vi "Translate front panels.vi"(7 "error in (no error)":errorcluster, 9 "Defer Panel Updates? (T)":bool=TRUE, 10 "Language":string) -> (0 "error out":errorcluster)   [LabVIEW 2019, in "Language Selection.lvlib"]
doc: "Translates the controls in the VI according to the translation settings\n- - -\nCopyright (c) 2026, Merecs Engineering GmbH"
uses:
  Language Selection.lvlib
  private/Global Language Selection.vi
panel:
  # "Connector Pane"
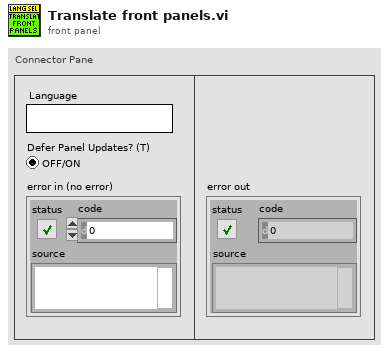
[diagram p1: front panel]
types:
  T1 = typedef "Language Selection.lvlib/Cluster Language Configuration.ctl" = cluster{"Data":T2, "Supported Languages":cluster{"ANSI":string[], "Unicode":string[]}, "VIs":path[], "FP Translations":T3[], "Text Translations":T3[]}
  T2 = typedef "Language Selection.lvlib/Cluster Settings Data.ctl" = cluster{"Startup Language":string, "Default Language":string, "Languages":cluster{"ANSI":string[], "Unicode":string[]}}
  T3 = typedef "Language Selection.lvlib/Cluster Language.ctl" = cluster{"Label":string, "Comment":string, "Property":T4[]}
  T4 = typedef "Language Selection.lvlib/Cluster PropertyTranslation.ctl" = cluster{"Type":T5, "Translation ANSI":string[], "Translation Unicode":string[]}
  T5 = typedef "Language Selection.lvlib/Enum Property Type.ctl" = enum16{"NA", "Caption", "String Value", "Boolean Text", "Ring Strings", "1D Array Elements", "2D Array Elements", "(MC)Listbox Header", "(MC)Listbox Items", "Tab Pages Names", "X & Y GraphChart", "Plot Names", "Table Headers", "Table Items", "TipStrip", "Combobox Strings", "Cursor Name", "Tree Col Headers"}
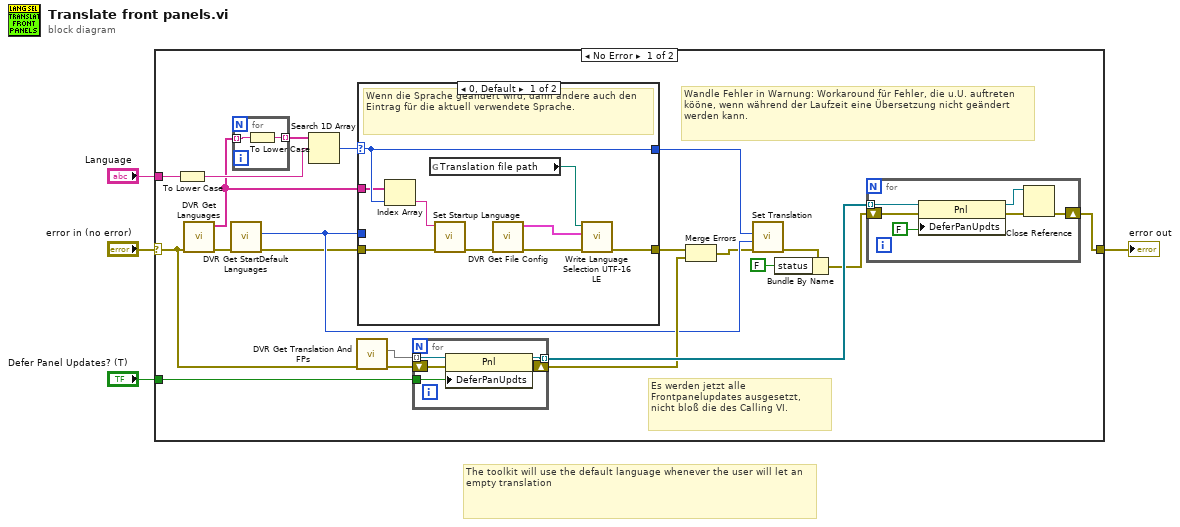
[diagram p0: block diagram]
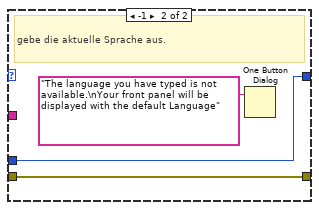
[diagram p2: hidden frame]
diagram:
  # "The toolkit will use the default language whenever the user will let an empty translation"
  n1 = case shown="No Error" "error in (no error)" {
    selector: "error in (no error)" -> [w10 w51]
    tunnel: [w18 w51] -> w3
    tunnel: "Language" -> [w23 _]
    tunnel: "Defer Panel Updates? (T)" -> [w19 _]
    frame No Error {
      # "Es werden jetzt alle Frontpanelupdates ausgesetzt, \nnicht bloß die des Calling VI."
      # "Wandle Fehler in Warnung: Workaround für Fehler, die u.U. auftreten kööne, wenn während der Laufzeit eine Übersetzung nicht geändert werden kann."
      n2 = To Lower Case(string=w23) -> (all lower case string=w22:string)
      n3 = call "DVR Get Languages.vi"("error in (no error)"=w10) -> ("error out"=w12:errorcluster, "Languages"=w14:string[])  [unwired: 7 in, 2 out]
      n4 = call "DVR Get StartDefault Languages.vi"("error in (no error)"=w12) -> ("error out"=w11:errorcluster, "Default"=w13:i32)  [unwired: 8 in, 1 out]
      n5 = for {
        tunnel: w14 -> [w38] mode=indexing
        tunnel: [w37] -> w21 mode=indexing
        n6 = To Lower Case(string=w38) -> (all lower case string=w37:string)
      }
      n7 = Search 1D Array(1D array=w21, element=w22) -> (index of element=w24:i32)  [unwired: 1 in]
      n8 = call "DVR Get Translation And FPs.vi"("error in (no error)"=w10) -> ("error out"=w15:errorcluster, "Front panels"=w16:set{refnum<vi>})  [unwired: 8 in, 1 out]
      n9 = case shown="0, Default" w24 {
        selector: w24 -> [w47 _]
        tunnel: [w47 w48] -> w20
        tunnel: w11 -> [w45 w50]
        tunnel: [w43 w50] -> w8
        tunnel: w14 -> [w46 _]
        tunnel: w13 -> [_ w48]
        frame 0, Default {
          # "Wenn die Sprache geändert wird, dann ändere auch den Eintrag für die aktuell verwendete Sprache."
          n10 = Index Array(array=w46, index=w47) -> (element=w44:string)
          n11 = global read "Global Language Selection.vi" "Translation file path"() -> (w39:path)
          n12 = call "Set Startup Language.vi"("error in (no error)"=w45, "Data.Startup Language"=w44) -> ("error out"=w42:errorcluster)  [unwired: 9 in]
          n13 = call "DVR Get File Config.vi"("error in (no error)"=w42) -> ("error out"=w41:errorcluster, "Config"=w40:T1)  [unwired: 9 in]
          n14 = call "Write Language Selection UTF-16 LE.vi"("error in (no error)"=w41, "Langúage Selection"=w40, "LanguageSelection file"=w39) -> ("error out"=w43:errorcluster)  [unwired: 7 in, 1 out]
        }
        frame -1 {
          # "gebe die aktuelle Sprache aus."
          n15 = One Button Dialog(message="The language you have typed is not available.\nYour front panel will be displayed with the default Language") -> ()  [unwired: 1 in, 1 out]
        }
      }
      n16 = for {
        tunnel: w16 -> [w36] mode=indexing
        tunnel: w19 -> [w35]
        tunnel: [w34] -> w25 mode=indexing
        shift-right: [w32] -> w17
        shift-left: w15 -> [w33]
        n17 = property class="Pnl"(reference=w36, error in=w33, "DeferPanUpdts"=w35) -> (reference out=w34:refnum<vi>, error out=w32:errorcluster)
      }
      n18 = Merge Errors(w8, w17) -> (w9:errorcluster)
      n19 = call "Set Translation.vi"("error in (no error)"=w9, "Default Lang"=w13, "Language"=w20) -> ("error out"=w7:errorcluster)  [unwired: 8 in]
      n20 = Bundle By Name(cluster=w7, "status"=FALSE) -> (w6:errorcluster)
      n21 = for {
        tunnel: w25 -> [w28] mode=indexing
        shift-right: [w26] -> w18
        shift-left: w6 -> [w27]
        n22 = property class="Pnl"(reference=w28, error in=w27, "DeferPanUpdts"=FALSE ("Defer Panel Updates")) -> (reference out=w29:refnum<vi>, error out=w30:errorcluster)
        n23 = Close Reference(reference=w29, error in (no error)=w30) -> (error out=w26:errorcluster)
      }
    }
    frame Error {
    }
  }
  "error out" <- w3
